vi "ScanRevised_Shane_Attepmt1.vi"() -> ()   [LabVIEW 2023, in "HP4192A IA.lvclass"]
uses:
  HP4192A IA.lvclass
  Global/GPIB Numbers.vi
  HP4192A Impedance Analyzer/HP4192 Impedance Analyzer.lvlib
  <vilib>/Analysis/NI_AALBase.lvlib
  <vilib>/Analysis/baseanly.llb/Mean (DBL).vi
  Global/Relative Sound Files.vi
  <vilib>/Utility/file.llb/Write Delimited Spreadsheet (DBL).vi
panel:
  in  "Tab Control":enum32{"Z", "R", "L", "C"}(tab)
  out "Impedance":cluster{"Y":dbl[], "Y":dbl[]}[](graph)=[{"Y"=[5.0, 5.0, 5.0, 5.0, 5.0], "Y"=[-246999.99999999997, -1063000.0, -361000.0, -401000.0, -539000.0]}]
  out "Resistance":cluster{"Y":dbl[], "Y":dbl[]}[](graph)=[{"Y"=[5.0, 5.0, 5.0, 5.0, 5.0], "Y"=[-246999.99999999997, -1063000.0, -361000.0, -401000.0, -539000.0]}]
  out "Inductance":cluster{"Y":dbl[], "Y":dbl[]}[](graph)=[{"Y"=[5.0, 5.0, 5.0, 5.0, 5.0], "Y"=[-246999.99999999997, -1063000.0, -361000.0, -401000.0, -539000.0]}]
  out "Capacitance":cluster{"Y":dbl[], "Y":dbl[]}[](graph)=[{"Y"=[5.0, 5.0, 5.0, 5.0, 5.0], "Y"=[-246999.99999999997, -1063000.0, -361000.0, -401000.0, -539000.0]}]
  out "Boolean 4":bool
  out "Boolean 3":bool
  out "Boolean 2":bool
  out "Boolean":bool
  in  "Numeric":i32=1
  out "dataTxt":string
  in  "Export\nPlot":bool
  in  "path":path
  out "error out":errorcluster
  in  "error in":errorcluster
  in  "Notes":string
  out "current numpoints":dbl
  in  "Take additional samples?":bool
  in  "number of samples in this range":i32=101
  in  "end freq for add'l sample":dbl[unit]=13000000.0
  in  "start freq for add'l samples":dbl[unit]=5.0
  in  "Total number of freq points":dbl=101.0
  in  "Final frequency":dbl[unit]=13000000.0
  in  "Initial frequency":dbl[unit]=5.0
  in  "Averaging?":bool
  in  "stop":bool
  out "Current Frequency":dbl[unit]
  in  "start":bool
  in  "L":bool
  in  "C":bool
  in  "R":bool
  in  "Z":bool
  # "Measure"
  # "Frequency range for additional samples"
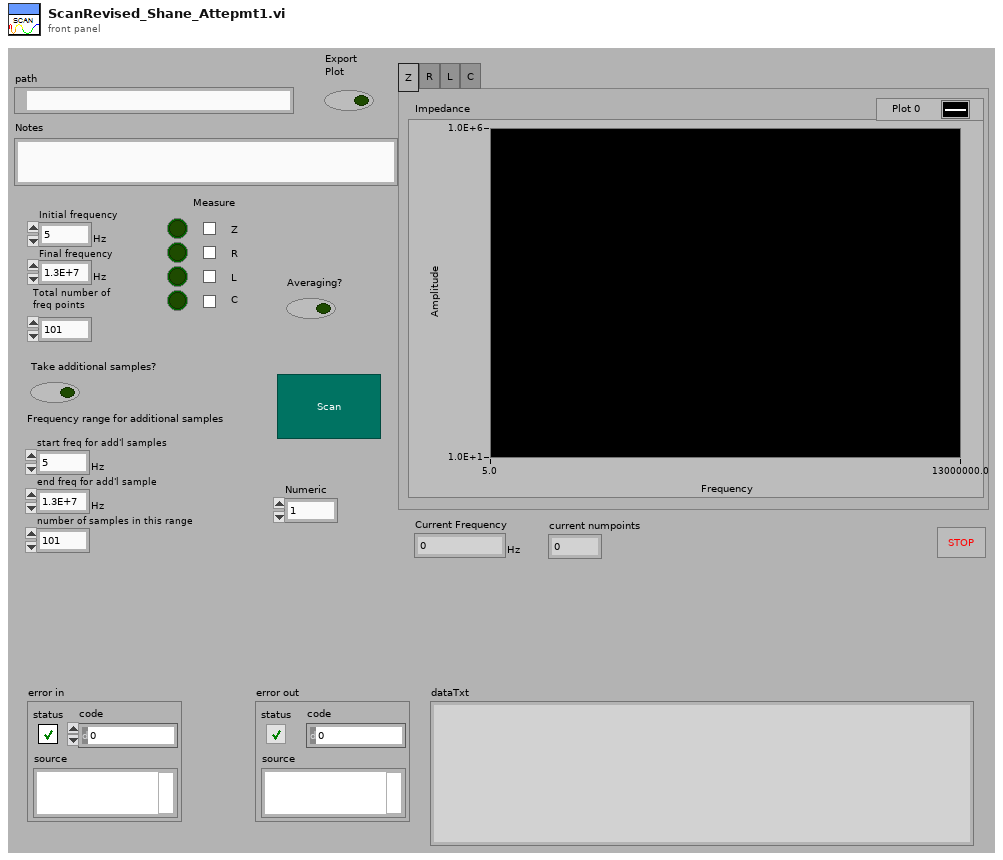
[diagram p1: front panel]
types:
  T1 = typedef "GPIB Type Def.ctl" = cluster{"Name":string, "bus":dbl, "GPIB":dbl, "GPIB as string":string, "byte":i32, "VISA Resource Name":refnum<visa-resource-name>}
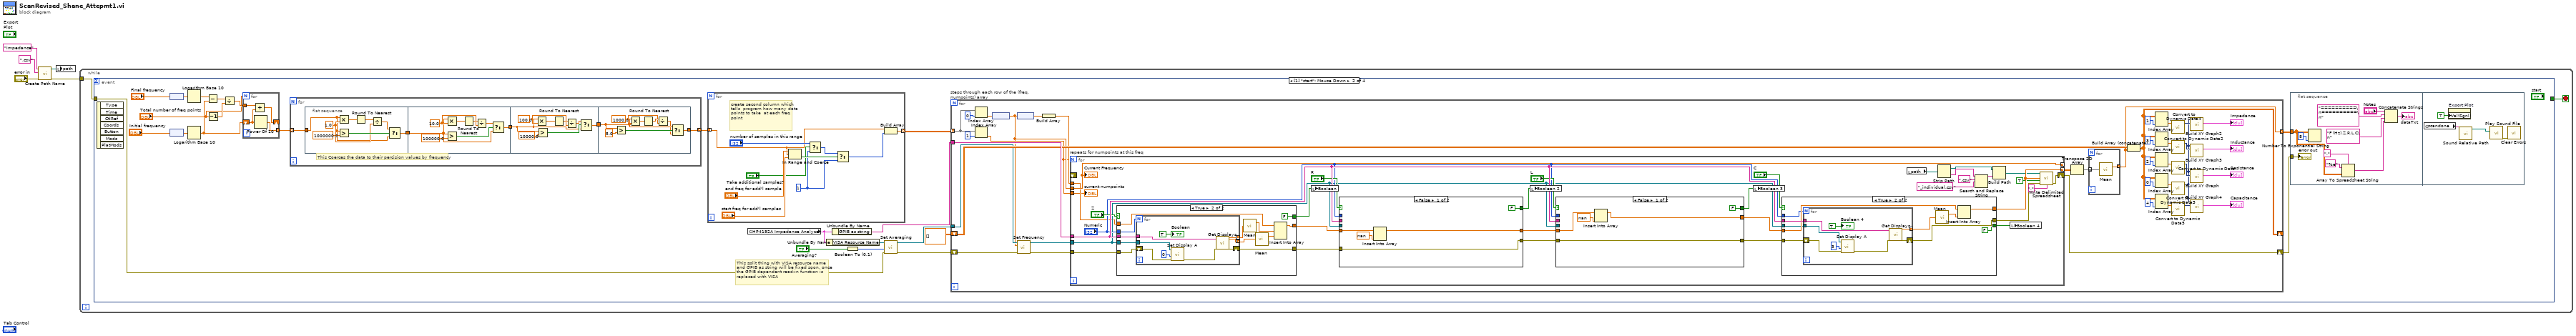
[diagram p0: block diagram]
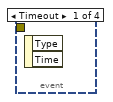
[diagram p2: hidden frame]
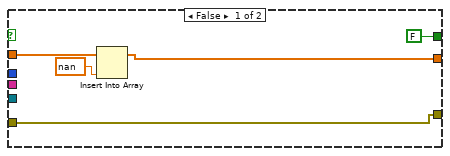
[diagram p3: hidden frame]
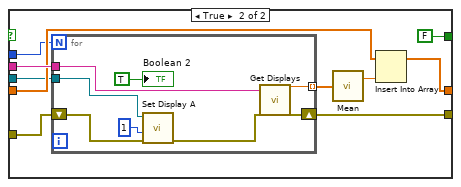
[diagram p4: hidden frame]
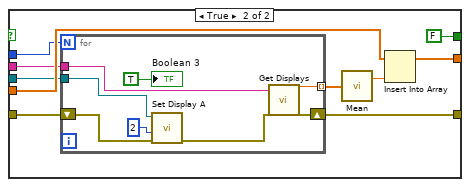
[diagram p5: hidden frame]
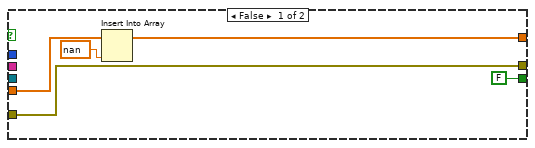
[diagram p6: hidden frame]
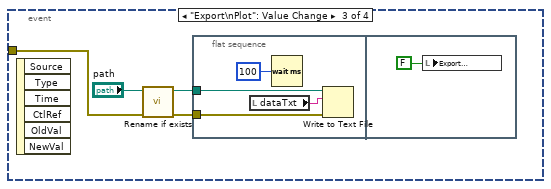
[diagram p7: hidden frame]
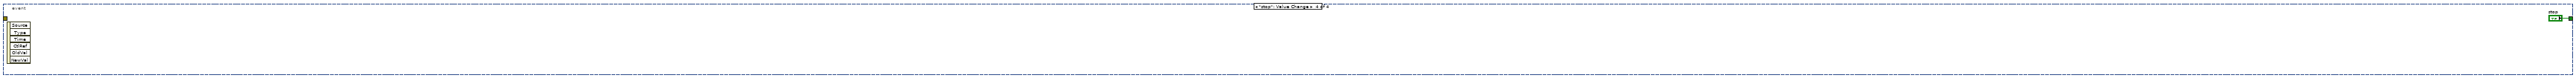
[diagram p8: hidden frame]
diagram:
  n1 = call "Create Path Name.vi"("error in"="error in", "String"=".csv", "filename"="impedance") -> ("error out"=w2:errorcluster, "path"=w4:path)  [unwired: 3 out]
  n2 = local write "path"(w4) -> ()
  n3 = while {
    tunnel: w2 -> [w6]
    stop <- w7 stop-if-true
    n4 = event shown="[1] \"start\": Mouse Down" {
      selector: _ -> [_ _ _ _]
      dyn-events: _ -> [_ _ _ _]
      timeout: _ -> [_ _ _ _]
      tunnel: [_ _ _ "stop"] -> w7
      tunnel: w6 -> [_ w11 w267 _]
      event Timeout {
        n5 = event-data() -> ()  [unwired: 1 in, 2 out]
      }
      event "start": Mouse Down {
        # "This split thing with VISA resource name  \nand GPIB as string will be fixed soon, once\nthe GPIB dependent read-in function is\nreplaced with VISA"
        n6 = event-data() -> ()  [unwired: 1 in, 7 out]
        n7 = node("Final frequency") -> (w19:dbl)
        n8 = node("Initial frequency") -> (w21:dbl)
        n9 = Logarithm Base 10(1:w19) -> (0:w26:dbl)
        n10 = Logarithm Base 10(1:w21) -> (0:w25:dbl)
        n11 = Subtract(x=w26, y=w25) -> (x-y=w31:dbl)
        n12 = Decrement(x="Total number of freq points") -> (x-1=w24:dbl)
        n13 = Divide(x=w31, y=w24) -> (x/y=w30:dbl)
        n14 = for {
          N: "Total number of freq points" -> [_]
          shift-right: [w264] -> _
          shift-left: w25 -> [w262]
          tunnel: w30 -> [w263]
          tunnel: [w261] -> w9 mode=indexing
          n15 = Add(x=w263, y=w262) -> (x+y=w264:dbl)
          n16 = Power Of 10(x=w262) -> (10^x=w261:dbl)
        }
        n17 = for {
          tunnel: w9 -> [w36] mode=indexing
          tunnel: [w35] -> w8 mode=indexing
          # "This Coerces the data to their percision values by frequency"
          n18 = flat-sequence {
            tunnel: w36 -> [w38]
            tunnel: [w37] -> w34
            tunnel: w34 -> [w46]
            tunnel: [w45] -> w33
            tunnel: w33 -> [w54]
            tunnel: [w53] -> w32
            tunnel: [w61] -> w35
            tunnel: w32 -> [w62]
            frame #0 {
              w41 = 1.0 ("y")
              n19 = Multiply(x=w38, y=w41) -> (x*y=w42:dbl)
              n20 = Greater?(x=w38, y=1000000.0) -> (0:w43:bool)
              n21 = Round To Nearest(number=w42) -> (nearest integer value=w40:dbl)
              n22 = Divide(x=w40, y=w41) -> (x/y=w39:dbl)
              n23 = Select(t=w39, s=w43, f=w38) -> (s? t:f=w37:dbl)
            }
            frame #1 {
              w47 = 10.0 ("y")
              n24 = Multiply(x=w46, y=w47) -> (x*y=w50:dbl)
              n25 = Greater?(x=w46, y=100000.0) -> (0:w49:bool)
              n26 = Round To Nearest(number=w50) -> (nearest integer value=w51:dbl)
              n27 = Divide(x=w51, y=w47) -> (x/y=w52:dbl)
              n28 = Select(t=w52, s=w49, f=w46) -> (s? t:f=w45:dbl)
            }
            frame #2 {
              w55 = 100.0 ("y")
              n29 = Multiply(x=w54, y=w55) -> (x*y=w58:dbl)
              n30 = Greater?(x=w54, y=10000.0) -> (0:w57:bool)
              n31 = Round To Nearest(number=w58) -> (nearest integer value=w59:dbl)
              n32 = Divide(x=w59, y=w55) -> (x/y=w60:dbl)
              n33 = Select(t=w60, s=w57, f=w54) -> (s? t:f=w53:dbl)
            }
            frame #3 {
              w63 = 1000.0 ("y")
              n34 = Greater?(x=w62, y=5.0) -> (0:w65:bool)
              n35 = Multiply(x=w62, y=w63) -> (x*y=w66:dbl)
              n36 = Round To Nearest(number=w66) -> (nearest integer value=w67:dbl)
              n37 = Divide(x=w67, y=w63) -> (x/y=w68:dbl)
              n38 = Select(t=w68, s=w65, f=w62) -> (s? t:f=w61:dbl)
            }
          }
        }
        n39 = for {
          tunnel: w8 -> [w251] mode=indexing
          tunnel: [w252] -> w18 mode=indexing
          w255 = 1 ("f")
          # "create second column which tells  program how many data points to take  at each freq point"
          n40 = In Range and Coerce(upper limit="end freq for add'l sample", x=w251, lower limit="start freq for add'l samples") -> (In Range?=w258:bool)  [unwired: 1 out]
          n41 = Select(t="number of samples in this range", s="Take additional samples?", f=w255) -> (s? t:f=w254:i32)
          n42 = Select(t=w254, s=w258, f=w255) -> (s? t:f=w253:i32)
          n43 = Build Array(w251, w253) -> (w252:dbl[])
        }
        n44 = global read "GPIB Numbers.vi" "HP4192A Impedance Analyzer"() -> (w27:T1)
        n45 = Unbundle By Name(w27) -> ("VISA Resource Name"=w28:refnum<visa-resource-name>)
        n46 = Unbundle By Name(w27) -> ("GPIB as string"=w29:string)
        n47 = Boolean To (0,1)(Boolean="Averaging?") -> (0, 1=w15:i16)
        n48 = call "Set Averaging.vi"("error in (no error)"=w11, "Averaging"=w15, "VISA resource name"=w28) -> ("error out"=w13:errorcluster, "VISA resource name out"=w14:refnum<visa-resource-name>)  [unwired: 7 in]
        n49 = for "steps through each row of the (freq, numpoints) array" {
          tunnel: w18 -> [w110] mode=indexing
          tunnel: w29 -> [w120]
          tunnel: [w105] -> w10 mode=indexing
          shift-right: [w94] -> _
          shift-left: dbl[][] [] -> [w119]
          tunnel: w14 -> [w118]
          shift-right: [w84] -> w12
          shift-left: w13 -> [w90]
          n50 = Index Array(array=w110, index=0) -> (element=w108:dbl)
          n51 = Index Array(array=w110, index=1) -> (element=w85:dbl)
          n52 = node(w108) -> (w107:dbl[unit])
          n53 = node(w107) -> (w86:dbl)
          n54 = call "Set Frequency.vi"("error in (no error)"=w90, "test signal freq"=w107, "VISA resource name"=w118) -> ("error out"=w89:errorcluster, "VISA resource name out"=w88:refnum<visa-resource-name>)  [unwired: 7 in]
          n55 = Build Array(w86) -> (w87:dbl[])
          n56 = for "repeats for numpoints at this freq" {
            N: w85 -> [_]
            tunnel: w120 -> [w155]
            tunnel: w107 -> [w154]
            tunnel: [w134] -> w83 mode=indexing
            shift-right: [w132] -> w84
            shift-left: _ -> [_]
            tunnel: [w154] -> _ mode=indexing
            tunnel: w89 -> [w138]
            tunnel: w88 -> [w137]
            tunnel: w87 -> [w136]
            tunnel: w85 -> [w135]
            n57 = case shown="True" "Z" {
              tunnel: w136 -> [w158 w171]
              tunnel: w155 -> [_ w172]
              tunnel: [w157 w170] -> w147
              tunnel: w137 -> [_ w167]
              tunnel: w138 -> [w160 w168]
              tunnel: [w160 w166] -> w144
              tunnel: "Numeric" -> [_ w165]
              tunnel: [FALSE ("Boolean") FALSE ("Boolean")] -> w142
              frame False {
                n58 = Insert Into Array(array=w158, new element=nan) -> (w157:dbl[])  [unwired: 1 in]
              }
              frame True {
                n59 = for {
                  N: w165 -> [_]
                  tunnel: w172 -> [w181]
                  tunnel: [w180] -> w169 mode=indexing
                  tunnel: w167 -> [w178]
                  shift-right: [w176] -> w166
                  shift-left: w168 -> [w179]
                  tunnel: [w173] -> w162 mode=indexing
                  n60 = call "Set Display A.vi"("error in (no error)"=w179, "function A (z/y:0)"=i16 0, "VISA resource name"=w178) -> ("error out 2"=w177:errorcluster)  [unwired: 8 in]
                  n61 = call "Get Displays.vi"("GPIB addess"=w181, "error in (no error)"=w177) -> ("display A"=w180:dbl, "display B"=w173:dbl, "error out"=w176:errorcluster)  [unwired: 17 in, 6 out]
                  "Boolean" <- TRUE ("Boolean")
                }
                n62 = call-poly <vilib>:"Mean.vi"("X"=w169) -> ("mean"=w163:dbl)  [unwired: 1 out]
                n63 = call-poly <vilib>:"Mean.vi"("X"=w162) -> ("mean"=w161:dbl)  [unwired: 1 out]
                n64 = Insert Into Array(array=w171, new element #1=w163, new element #2=w161) -> (w170:dbl[])  [unwired: 1 in]
              }
            }
            n65 = local write "Boolean"(w142) -> ()
            n66 = case shown="False" "R" {
              tunnel: w155 -> [_ w196]
              tunnel: w147 -> [w182 w195]
              tunnel: [w183 w194] -> w150
              tunnel: w137 -> [_ w193]
              tunnel: w144 -> [w186 w192]
              tunnel: [w186 w191] -> w148
              tunnel: "Numeric" -> [_ w188]
              tunnel: [FALSE ("Boolean 2") FALSE ("Boolean 2")] -> w141
              frame False {
                n67 = Insert Into Array(array=w182, new element=nan ("new element/subarray")) -> (w183:dbl[])  [unwired: 1 in]
              }
              frame True {
                n68 = for {
                  N: w188 -> [_]
                  tunnel: [w204] -> w190 mode=indexing
                  tunnel: w196 -> [w203]
                  tunnel: w193 -> [w202]
                  shift-right: [w199] -> w191
                  shift-left: w192 -> [w201]
                  n69 = call "Set Display A.vi"("error in (no error)"=w201, "function A (z/y:0)"=i16 1, "VISA resource name"=w202) -> ("error out 2"=w200:errorcluster)  [unwired: 8 in]
                  n70 = call "Get Displays.vi"("GPIB addess"=w203, "error in (no error)"=w200) -> ("display A"=w204:dbl, "error out"=w199:errorcluster)  [unwired: 17 in, 7 out]
                  "Boolean 2" <- TRUE ("Boolean 2")
                }
                n71 = call-poly <vilib>:"Mean.vi"("X"=w190) -> ("mean"=w189:dbl)  [unwired: 1 out]
                n72 = Insert Into Array(array=w195, new element=w189) -> (w194:dbl[])  [unwired: 1 in]
              }
            }
            n73 = local write "Boolean 2"(w141) -> ()
            n74 = case shown="False" "L" {
              tunnel: [w206 w219] -> w153
              tunnel: w150 -> [w207 w218]
              tunnel: w155 -> [_ w217]
              tunnel: w137 -> [_ w216]
              tunnel: w148 -> [w209 w215]
              tunnel: [w209 w214] -> w151
              tunnel: "Numeric" -> [_ w211]
              tunnel: [FALSE ("Boolean 3") FALSE ("Boolean 3")] -> w140
              frame False {
                n75 = Insert Into Array(array=w207, new element=nan) -> (w206:dbl[])  [unwired: 1 in]
              }
              frame True {
                n76 = for {
                  N: w211 -> [_]
                  tunnel: [w227] -> w213 mode=indexing
                  tunnel: w217 -> [w226]
                  tunnel: w216 -> [w225]
                  shift-right: [w222] -> w214
                  shift-left: w215 -> [w224]
                  n77 = call "Set Display A.vi"("error in (no error)"=w224, "function A (z/y:0)"=i16 2, "VISA resource name"=w225) -> ("error out 2"=w223:errorcluster)  [unwired: 8 in]
                  n78 = call "Get Displays.vi"("GPIB addess"=w226, "error in (no error)"=w223) -> ("display A"=w227:dbl, "error out"=w222:errorcluster)  [unwired: 17 in, 7 out]
                  "Boolean 3" <- TRUE ("Boolean 3")
                }
                n79 = call-poly <vilib>:"Mean.vi"("X"=w213) -> ("mean"=w212:dbl)  [unwired: 1 out]
                n80 = Insert Into Array(array=w218, new element=w212) -> (w219:dbl[])  [unwired: 1 in]
              }
            }
            n81 = local write "Boolean 3"(w140) -> ()
            n82 = case shown="True" "C" {
              tunnel: [w229 w242] -> w134
              tunnel: w155 -> [_ w241]
              tunnel: w153 -> [w230 w240]
              tunnel: w137 -> [_ w239]
              tunnel: w151 -> [w232 w238]
              tunnel: [w232 w237] -> w133
              tunnel: "Numeric" -> [_ w234]
              tunnel: [FALSE ("Boolean 3") FALSE ("Boolean 3")] -> w139
              frame False {
                n83 = Insert Into Array(array=w230, new element=nan) -> (w229:dbl[])  [unwired: 1 in]
              }
              frame True {
                n84 = for {
                  N: w234 -> [_]
                  tunnel: [w250] -> w236 mode=indexing
                  tunnel: w241 -> [w249]
                  tunnel: w239 -> [w248]
                  shift-right: [w245] -> w237
                  shift-left: w238 -> [w247]
                  n85 = call "Set Display A.vi"("error in (no error)"=w247, "function A (z/y:0)"=i16 3, "VISA resource name"=w248) -> ("error out 2"=w246:errorcluster)  [unwired: 8 in]
                  n86 = call "Get Displays.vi"("GPIB addess"=w249, "error in (no error)"=w246) -> ("display A"=w250:dbl, "error out"=w245:errorcluster)  [unwired: 17 in, 7 out]
                  "Boolean 4" <- TRUE ("Boolean 3")
                }
                n87 = call-poly <vilib>:"Mean.vi"("X"=w236) -> ("mean"=w235:dbl)  [unwired: 1 out]
                n88 = Insert Into Array(array=w240, new element=w235) -> (w242:dbl[])  [unwired: 1 in]
              }
            }
            n89 = local read "path"() -> (w131:path)
            n90 = Strip Path(path=w131) -> (stripped path=w127:path, name=w130:string)
            n91 = Search and Replace String(input string=w130, search string=".csv", replace string="_individual.csv" ("replace string (\"\")")) -> (result string=w126:string)  [unwired: 5 in, 3 out]
            n92 = Build Path(base path=w127, name or relative path=w126) -> (appended path=w125:path)
            n93 = local write "Boolean 4"(w139) -> ()
            n94 = call-poly <vilib>:"Write Delimited Spreadsheet.vi"("file path (dialog if empty)"=w125, "1D data"=w134, "append to file? (new file:F)"=TRUE, "error in (no error)"=w133, "delimiter (\\t)"="," ("delimiter (\\t)")) -> ("error out"=w132:errorcluster)  [unwired: 9 in, 1 out]
            "Current Frequency" <- w154
            "current numpoints" <- w135
          }
          n95 = Transpose 2D Array(2D array=w83) -> (transposed array=w106:dbl[][])
          n96 = for {
            tunnel: w106 -> [w122] mode=indexing
            tunnel: [w121] -> w105 mode=indexing
            n97 = call-poly <vilib>:"Mean.vi"("X"=w122) -> ("mean"=w121:dbl)  [unwired: 1 out]
          }
          n98 = Build Array (concatenate)(w119, w105) -> (w94:dbl[][])
          n99 = Index Array(array=w94, index (col)=1) -> (element=w112:dbl[])  [unwired: 1 in]
          n100 = Index Array(array=w94, index (col)=3) -> (element=w98:dbl[])  [unwired: 1 in]
          n101 = Index Array(array=w94, index (col)=2) -> (element=w102:dbl[])  [unwired: 1 in]
          n102 = Index Array(array=w94, index (col)=0) -> (element=w113:dbl[])  [unwired: 1 in]
          n103 = Index Array(array=w94, index (col)=4) -> (element=w95:dbl[])  [unwired: 1 in]
          n104 = call "Convert to Dynamic Data4"("Array"=w112) -> ("Dynamic Data Type"=w114:dynamicdata)  [unwired: 3 in]
          n105 = call "Convert to Dynamic Data2"("Array"=w98) -> ("Dynamic Data Type"=w99:dynamicdata)  [unwired: 3 in]
          n106 = call "Convert to Dynamic Data"("Array"=w102) -> ("Dynamic Data Type"=w103:dynamicdata)  [unwired: 3 in]
          n107 = call "Convert to Dynamic Data3"("Array"=w113) -> ("Dynamic Data Type"=w93:dynamicdata)  [unwired: 3 in]
          n108 = call "Convert to Dynamic Data5"("Array"=w95) -> ("Dynamic Data Type"=w96:dynamicdata)  [unwired: 3 in]
          n109 = call "Build XY Graph2"("Y Input"=w114, "X Input"=w93) -> ("XY Graph"=→"Impedance":cluster{"Y":dbl[], "Y":dbl[]}[])  [unwired: 8 in, 1 out]
          n110 = call "Build XY Graph3"("Y Input"=w99, "X Input"=w93) -> ("XY Graph"=→"Inductance":cluster{"Y":dbl[], "Y":dbl[]}[])  [unwired: 8 in, 1 out]
          n111 = call "Build XY Graph"("Y Input"=w103, "X Input"=w93) -> ("XY Graph"=→"Resistance":cluster{"Y":dbl[], "Y":dbl[]}[])  [unwired: 8 in, 1 out]
          n112 = call "Build XY Graph4"("Y Input"=w96, "X Input"=w93) -> ("XY Graph"=→"Capacitance":cluster{"Y":dbl[], "Y":dbl[]}[])  [unwired: 8 in, 1 out]
        }
        n113 = flat-sequence {
          tunnel: w12 -> [w78]
          tunnel: w10 -> [w70]
          frame #0 {
            n114 = Number To Exponential String(number=w70, precision (6)=i16 8) -> ()  [unwired: 2 in, 1 out]
            n115 = Array To Spreadsheet String(delimiter (Tab)=",", array=w70, 3:"%e") -> (spreadsheet string=w72:string)
            n116 = Concatenate Strings("Notes", "==========\n==========\n" ("string"), "F (Hz),Z,R,L,C\n", w72) -> (→"dataTxt":string)
            "error out" <- w78
          }
          frame #1 {
            n117 = global read "Relative Sound Files.vi" "scandone"() -> (w82:string)
            n118 = property on="Export Plot" class="Bool (strict)"("Val(Sgnl)"=TRUE ("Value (Signaling)")) -> ()  [unwired: 2 in, 2 out]
            n119 = call "Sound Relative Path.vi"("Sound"=w82) -> ("Relative Path"=w79:path)  [unwired: 10 in]
            n120 = call <vilib>:"Play Sound File.vi"("path"=w79) -> ("error out"=w81:errorcluster)  [unwired: 3 in, 7 out]
            n121 = call <vilib>:"Clear Errors.vi"("error in (no error)"=w81) -> ()  [unwired: 1 in, 6 out]
          }
        }
      }
      event "Export\nPlot": Value Change {
        n122 = event-data() -> ()  [unwired: 1 in, 6 out]
        n123 = call "Rename if exists.vi"("error in"=w267, "File Path"="path") -> ("error out"=w265:errorcluster, "New path"=w266:path)  [unwired: 1 in, 7 out]
        n124 = flat-sequence {
          tunnel: w266 -> [w271]
          tunnel: w265 -> [w270]
          frame #0 {
            n125 = local read "dataTxt"() -> (w272:string)
            n126 = Wait (ms)(milliseconds to wait=u32 100) -> ()  [unwired: 1 out]
            n127 = Write to Text File(file (use dialog)=w271, text=w272, error in=w270) -> ()  [unwired: 1 in, 3 out]
          }
          frame #1 {
            n128 = local write "Export\nPlot"(FALSE ("Export\nPlot")) -> ()
          }
        }
      }
      event "stop": Value Change {
        n129 = event-data() -> ()  [unwired: 1 in, 6 out]
      }
    }
  }
